vi "HostMem Swap.vi"(8 "error in (no error)":errorcluster, 10 "B in":refnum<class "HostMem.lvclass">, 11 "A in":refnum<class "HostMem.lvclass">) -> (0 "error out":errorcluster, 2 "B out":refnum<class "HostMem.lvclass">, 3 "A out":refnum<class "HostMem.lvclass">)   [LabVIEW 2020, in "OpenLvVision_OpenCv.lvlib" / "Cuda.lvlib" / "HostMem.lvclass"]
doc: "Swaps with other smart pointer"
uses:
  HostMem.lvclass
  C:/Users/lukas/Documents/OpenLvVision_OpenCv/SourceCode/LabView/OpenLvVision_OpenCv/_LvHelpers/EdvrObject/EdvrObject.lvclass
  _LvHelpers/EdvrObject/EdvrObject.lvclass/EdvrObject.ctl
  OpenLvVision_OpenCv.lvlib
  <vilib>/Utility/error.llb/Error Cluster From Error Code.vi
  <vilib>/ErrorRing/Error Ring.xnode
  _LvHelpers/EdvrObject/EdvrObject.lvclass
  Dlls/OlvOpenCvWrapper.dll
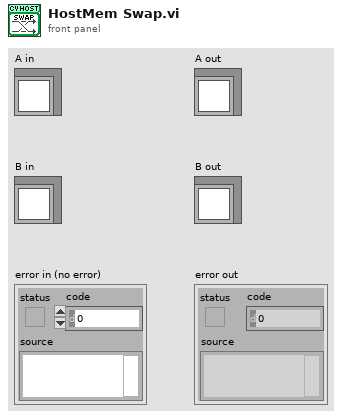
[diagram p1: front panel]
types:
  T1 = typedef "OpenLvVision_OpenCv.lvlib/EdvrObject.lvclass/Edvr.ctl" = refnum<data-value>
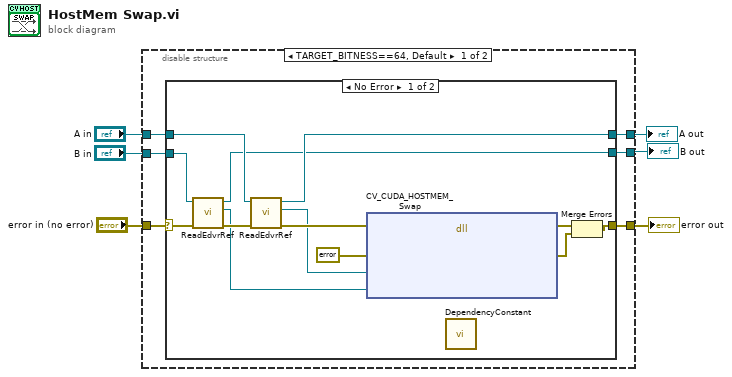
[diagram p0: block diagram]
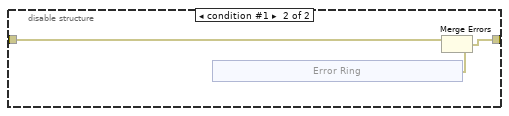
[diagram p3: hidden frame]
diagram:
  n1 = disable-structure shown="TARGET_BITNESS==64, Default" {
    disable-tunnel: "error in (no error)" -> [w12 w30]
    disable-tunnel: [w11 w31] -> w5
    disable-tunnel: "A in" -> [w10 _]
    disable-tunnel: [w9 _] -> w3
    disable-tunnel: "B in" -> [w8 _]
    disable-tunnel: [w7 _] -> w1
    frame condition #0 (active) {
      n2 = case shown="No Error" w12 {
        selector: w12 -> [w17 w28]
        tunnel: [w18 w28] -> w11
        tunnel: w10 -> [w22 w27]
        tunnel: [w19 w27] -> w9
        tunnel: w8 -> [w15 w26]
        tunnel: [w14 w26] -> w7
        frame No Error {
          n3 = call "ReadEdvrRef.vi"("error in (no error)"=w17, "EdvrObject in"=w15) -> ("error out"=w16:errorcluster, "Edvr"=w13:T1, "EdvrObject out"=w14:refnum<class "HostMem.lvclass">)  [unwired: 7 in]
          n4 = call "ReadEdvrRef.vi"("error in (no error)"=w16, "EdvrObject in"=w22) -> ("error out"=w21:errorcluster, "Edvr"=w20:T1, "EdvrObject out"=w19:refnum<class "HostMem.lvclass">)  [unwired: 7 in]
          n5 = dll-call lib="C:/Users/lukas/Documents/OpenLvVision_OpenCv/SourceCode/LabView/OpenLvVision_OpenCv/Dlls/OlvOpenCvWrapper.dll" fn="CV_CUDA_HOSTMEM_Swap"(error in=w21, "Error"=errorcluster {"status"=FALSE, "code"=0, "source"=""} ("error out"), "edvrRefA"=w20, "edvrRefB"=w13) -> (error out=w25:errorcluster, "Error"=w24:errorcluster)  [unwired: 5 in, 1 out]
          n6 = call "DependencyConstant.vi"() -> ()  [unwired: 12 in]
          n7 = Merge Errors(w25, w24) -> (w18:errorcluster)
        }
        frame Error {
        }
      }
    }
    frame condition #1 {
      n8 = xnode "Error Ring"() -> ("error out"=w29:errorcluster)
      n9 = Merge Errors(w30, w29) -> (w31:errorcluster)
    }
  }
  "error out" <- w5
  "A out" <- w3
  "B out" <- w1
